vi "check Device IDN.vi"(8 "error in":errorcluster, 10 "Spectrum Device Type":T1, 11 "VISA resource name":refnum<visa-resource-name>) -> (0 "error out":errorcluster, 1 "Connection Msg":string, 2 "Device name from IDN matched?":bool, 3 "Interface_Spectrum.lvclass":refnum<class "Interface_Spectrum.lvclass">)   [LabVIEW 2023, in "Spectrum Analyzer.lvlib"]
uses:
  Spectrum Analyzer.lvlib
  TYPE DEFINITION/TYPE Supported Spectrum Device Type.ctl
  Interface_Spectrum/Interface_Spectrum.lvclass
  Class/FSV-40N/FSV-40N.lvclass
  D:/Project/IST013_CE Conduction Measurement/IST013-CE-Condcuted-Measurement/src/Spectrum Analyzer/Interface_Spectrum/Interface_Spectrum.lvclass
  Class/FSV-40N/FSV-40N.lvclass/FSV-40N.ctl
  Class/Keysight 9020A/Keysight 9020A.lvclass
  Class/Keysight 9020A/Keysight 9020A.lvclass/Keysight 9020A.ctl
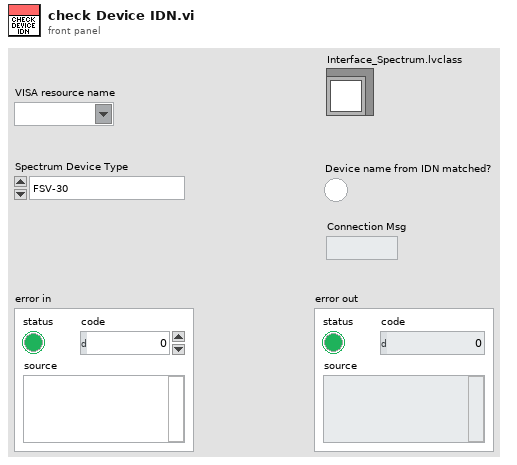
[diagram p1: front panel]
types:
  T1 = typedef "Spectrum Analyzer.lvlib/TYPE Supported Spectrum Device Type.ctl" = enum16{"FSV-30", "FSV-40", "9020A"}
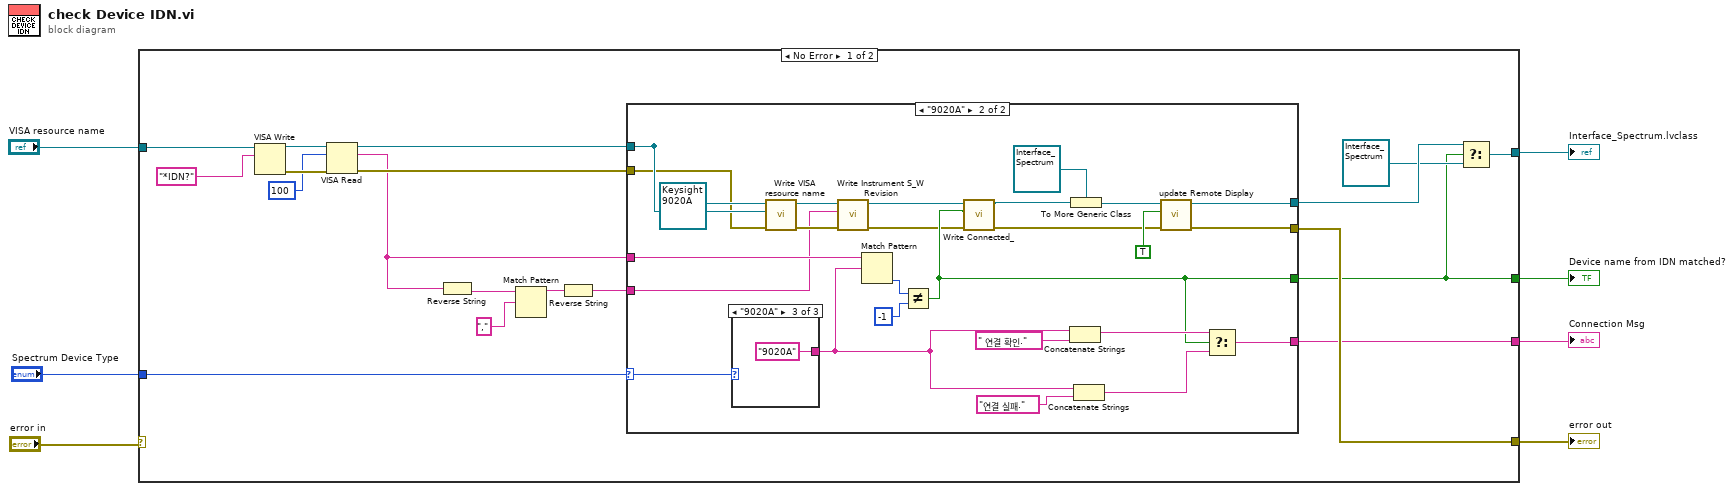
[diagram p0: block diagram]
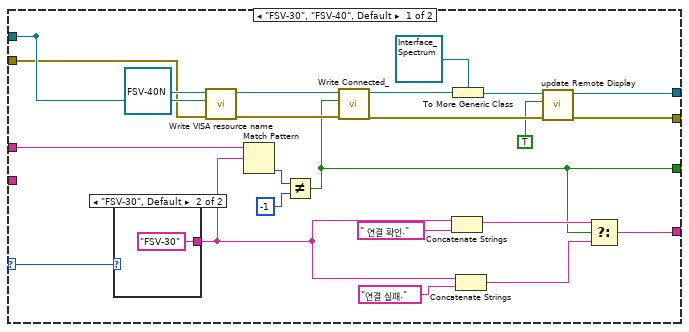
[diagram p2: hidden frame]
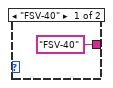
[diagram p3: hidden frame]
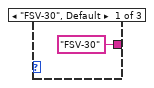
[diagram p4: hidden frame]
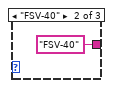
[diagram p5: hidden frame]
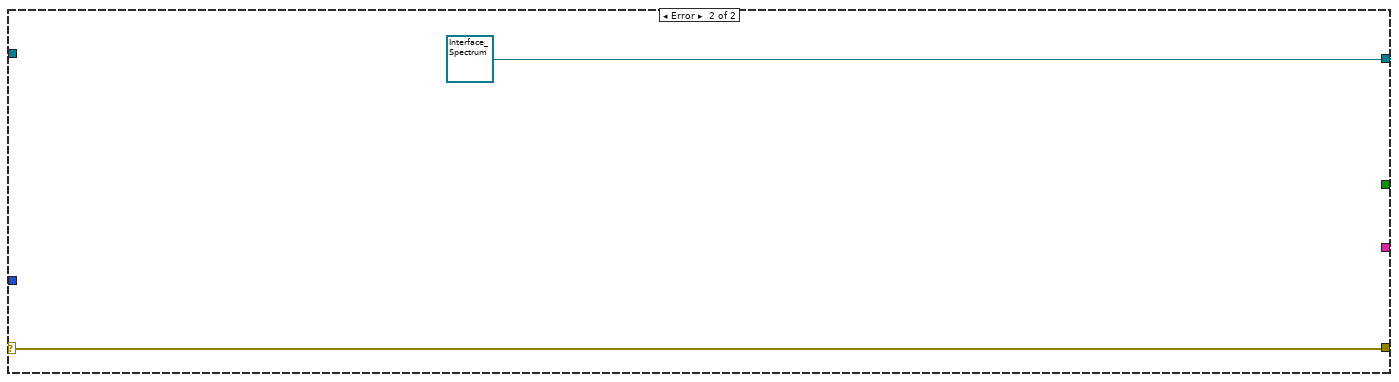
[diagram p6: hidden frame]
diagram:
  n1 = case shown="No Error" "error in" {
    selector: "error in" -> [_ w82]
    tunnel: "VISA resource name" -> [w26 _]
    tunnel: "Spectrum Device Type" -> [w25 _]
    tunnel: [w14 _] -> w4
    tunnel: [w18 refnum<class "Interface_Spectrum.lvclass"> refnum ("Spectrum Analyzer.lvlib:Interface_Spectrum.lvclass")] -> w3
    tunnel: [w15 w82] -> w2
    tunnel: [w13 _] -> w1
    frame No Error {
      n2 = VISA Write(VISA resource name=w26, write buffer="*IDN?") -> (VISA resource name out=w23:refnum<visa-resource-name>, error out=w22:errorcluster)  [unwired: 1 in, 1 out]
      n3 = VISA Read(VISA resource name=w23, byte count=u32 100, error in (no error)=w22) -> (VISA resource name out=w17:refnum<visa-resource-name>, read buffer=w9:string, error out=w16:errorcluster)  [unwired: 1 out]
      n4 = Reverse String(1:w9) -> (0:w12:string)
      n5 = Match Pattern(string=w12, regular expression=",") -> (before substring=w10:string)  [unwired: 1 in, 3 out]
      n6 = Reverse String(1:w10) -> (0:w8:string)
      n7 = case shown="\"9020A\"" w25 {
        selector: w25 -> [w28 w64]
        tunnel: [w36 w69] -> w13
        tunnel: [w32 w67] -> w20
        tunnel: [w47 w61] -> _
        tunnel: w17 -> [w47 w61]
        tunnel: w9 -> [w46 w76]
        tunnel: [w35 w59] -> w14
        tunnel: w16 -> [w34 w60]
        tunnel: [w30 w66] -> w15
        tunnel: w8 -> [_ w52]
        frame "FSV-30", "FSV-40", Default {
          n8 = case shown="\"FSV-30\", Default" w28 {
            tunnel: ["FSV-40" "FSV-30"] -> w27
            frame "FSV-40" {
            }
            frame "FSV-30", Default {
            }
          }
          n9 = call "Write VISA resource name.vi"("error in (no error)"=w34, "VISA resource name"=w47, "FSV-40N in"=refnum<class "FSV-40N.lvclass"> refnum ("Spectrum Analyzer.lvlib:FSV-40N.lvclass")) -> ("error out"=w42:errorcluster, "FSV-40N out"=w43:refnum<class "FSV-40N.lvclass">)  [unwired: 7 in]
          n10 = Match Pattern(string=w46, regular expression=w27) -> (offset past match=w44:i32)  [unwired: 1 in, 3 out]
          n11 = Not Equal?(x=w44, y=-1) -> (x != y?=w35:bool)
          n12 = call "Write Connected_.vi"("error in (no error)"=w42, "Connected?"=w35, "FSV-40N in"=w43) -> ("error out"=w31:errorcluster, "FSV-40N out"=w41:refnum<class "FSV-40N.lvclass">)  [unwired: 7 in]
          n13 = Concatenate Strings(w27, " 연결 확인." ("string")) -> (w39:string)
          n14 = To More Generic Class(target class=refnum<class "Interface_Spectrum.lvclass"> refnum ("Spectrum Analyzer.lvlib:Interface_Spectrum.lvclass"), reference=w41) -> (generic class reference=w33:refnum<class "Interface_Spectrum.lvclass">)
          n15 = Concatenate Strings(w27, "연결 실패." ("string")) -> (w37:string)
          n16 = call-dynamic "update Remote Display.vi"("error in (no error)"=w31, "Remote Display On?"=TRUE, "Interface_Spectrum in"=w33) -> ("error out"=w30:errorcluster, "Interface_Spectrum out"=w32:refnum<class "Interface_Spectrum.lvclass">)  [unwired: 7 in]
          n17 = Select(t=w39, s=w35, f=w37) -> (s? t:f=w36:string)
        }
        frame "9020A" {
          n18 = case shown="\"9020A\"" w64 {
            tunnel: ["FSV-30" "FSV-40" "9020A"] -> w63
            frame "FSV-30", Default {
            }
            frame "FSV-40" {
            }
            frame "9020A" {
            }
          }
          n19 = call "Write VISA resource name.vi"("error in (no error)"=w60, "VISA resource name"=w61, "Keysight 9020A in"=refnum<class "Keysight 9020A.lvclass"> refnum ("Spectrum Analyzer.lvlib:Keysight 9020A.lvclass")) -> ("error out"=w55:errorcluster, "Keysight 9020A out"=w56:refnum<class "Keysight 9020A.lvclass">)  [unwired: 7 in]
          n20 = call "Write Instrument S_W Revision.vi"("error in (no error)"=w55, "Instrument S/W Revision"=w52, "Keysight 9020A in"=w56) -> ("error out"=w53:errorcluster, "Keysight 9020A out"=w54:refnum<class "Keysight 9020A.lvclass">)  [unwired: 7 in]
          n21 = Match Pattern(string=w76, regular expression=w63) -> (offset past match=w74:i32)  [unwired: 1 in, 3 out]
          n22 = Not Equal?(x=w74, y=-1) -> (x != y?=w59:bool)
          n23 = call "Write Connected_.vi"("error in (no error)"=w53, "Connected?"=w59, "Keysight 9020A in"=w54) -> ("error out"=w57:errorcluster, "Keysight 9020A out"=w58:refnum<class "Keysight 9020A.lvclass">)  [unwired: 7 in]
          n24 = Concatenate Strings(w63, " 연결 확인." ("string")) -> (w72:string)
          n25 = To More Generic Class(target class=refnum<class "Interface_Spectrum.lvclass"> refnum ("Spectrum Analyzer.lvlib:Interface_Spectrum.lvclass"), reference=w58) -> (generic class reference=w68:refnum<class "Interface_Spectrum.lvclass">)
          n26 = Concatenate Strings(w63, "연결 실패." ("string")) -> (w70:string)
          n27 = call-dynamic "update Remote Display.vi"("error in (no error)"=w57, "Remote Display On?"=TRUE, "Interface_Spectrum in"=w68) -> ("error out"=w66:errorcluster, "Interface_Spectrum out"=w67:refnum<class "Interface_Spectrum.lvclass">)  [unwired: 7 in]
          n28 = Select(t=w72, s=w59, f=w70) -> (s? t:f=w69:string)
        }
      }
      n29 = Select(t=w20, s=w14, f=refnum<class "Interface_Spectrum.lvclass"> refnum ("Spectrum Analyzer.lvlib:Interface_Spectrum.lvclass")) -> (s? t:f=w18:refnum<class "Interface_Spectrum.lvclass">)
    }
    frame Error {
    }
  }
  "error out" <- w2
  "Device name from IDN matched?" <- w4
  "Interface_Spectrum.lvclass" <- w3
  "Connection Msg" <- w1
